vi "Editor UI.vi"(10 "Close Event":refnum<user-event>, 11 "Device in":refnum<class "Device.lvclass">) -> ()   [LabVIEW 2020, in "HAL.lvlib" / "Device.lvclass"]
uses:
  Device.lvclass
  Editor Event Data.ctl
panel:
  # "No\nExtra\nConfig"
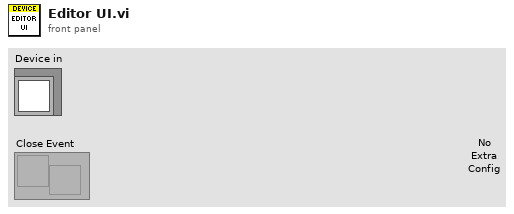
[diagram p1: front panel]
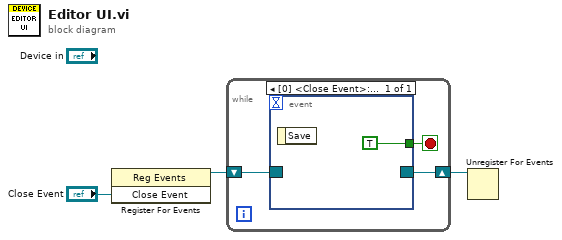
[diagram p0: block diagram]
diagram:
  n1 = register-events("Close Event") -> (reference out=w2:refnum<event-registration>)  [unwired: 2 in, 1 out]
  n2 = while {
    shift-right: [w5] -> w1
    shift-left: w2 -> [w6]
    stop <- w4 stop-if-true
    n3 = event shown="[0] <Close Event>: User Event" {
      selector: w6 -> [_]
      dyn-events: [_] -> w5
      timeout: _ -> [_]
      tunnel: [TRUE] -> w4
      event User Event {
        n4 = event-data() -> ()  [unwired: 1 in, 1 out]
      }
    }
  }
  n5 = Unregister For Events(event registration refnum=w1) -> ()  [unwired: 1 in, 1 out]
